vi "RDV-handle-AnalysePermittivityError.vi"(7 "%?":bool, 9 "set":i32, 10 "Reference key":string, 11 "RDV-Reflection_Data_viewer in":refnum<class "RDV-Reflection_Data_viewer.lvclass">) -> (0 "imag Error":dbl[](array[numeric]), 1 "imag":cluster{"Frequency":dbl[], "Perm 2":dbl[]}[](array[cluster]), 2 "real error":dbl[](array[numeric]), 3 "Real":cluster{"Frequency":dbl[], "Perm":dbl[]}[](array[cluster]))   [LabVIEW 2020, in "RDV-Reflection_Data_viewer.lvclass"]
doc: "Compares the permittivity of one data set in the viewer's map with the reference key, using RDC-permittivity-error_analysis. Returns the real and imaginary values and errors, as percent when %? is true."
uses:
  RDV-Reflection_Data_viewer.lvclass
  Computation/RDC-perm_calc_type.ctl
  RDV-Reflection_Data_viewer.lvclass/RDV-Reflection_Data_viewer.ctl
  Computation/RDC-Reflection_Data_Computation.lvlib
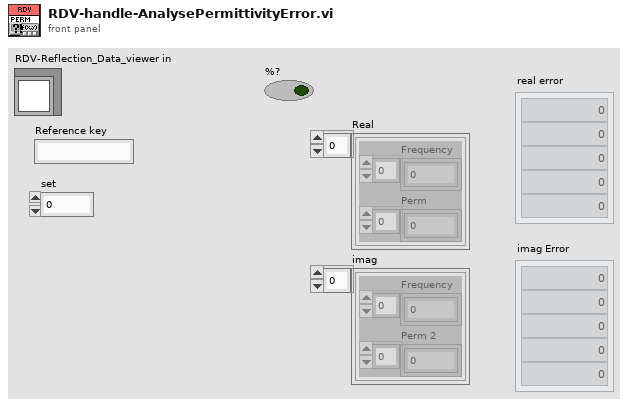
[diagram p1: front panel]
types:
  T1 = typedef "RDC-Reflection_Data_Computation.lvlib/RDC-perm_calc_type.ctl" = enum16{"Basic", "Capacative", "Advance", "Bilinear", "Size"}
  T2 = typedef "RDV-Reflection_Data_viewer.lvclass/RDV-UPDATE_IGNORE_LIST.ctl" = string[]
  T3 = typedef "RDV-Reflection_Data_viewer.lvclass/RDV-DATA_MAP.ctl" = map{string, T4}
  T4 = typedef "RDV-Reflection_Data_viewer.lvclass/RDV-DATA_MAP_CLUST.ctl" = cluster{"filename w/ ext":string, "Common Format":T5}
  T5 = typedef "RFH-Reflection_File_Handler.lvlib/RFH-common_data_format.ctl" = cluster{"Frequency":dbl[], "Reflection'":dbl[], "Reflection''":dbl[], "Permativity'":dbl[], "Permativity''":dbl[], "Conductivity":dbl[], "Loss Tangent":dbl[], "Resistance":dbl[], "Reactance":dbl[]}
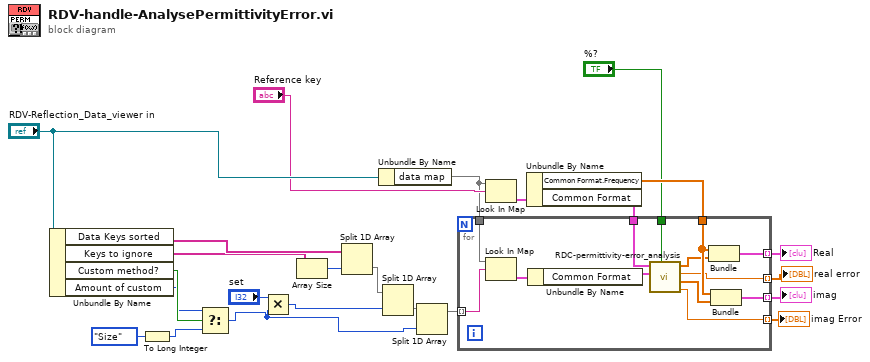
[diagram p0: block diagram]
diagram:
  n1 = Unbundle By Name("RDV-Reflection_Data_viewer in") -> ("Data Keys sorted"=w17:string[], "Keys to ignore"=w16:T2, "Custom method?"=w3:bool, "Amount of custom"=w2:i32)
  n2 = To Long Integer(number=RDC-perm_calc_type."Size" ("Perm calc type")) -> (32bit integer=w4:i32)
  n3 = Select(t=w2, s=w3, f=w4) -> (s? t:f=w1:i32)
  n4 = Multiply(x="set", y=w1) -> (x*y=w14:i32)
  n5 = Array Size(array=w16) -> (size(s)=w15:i32)
  n6 = Split 1D Array(array=w17, index=w15) -> (second subarray=w13:string[])  [unwired: 1 out]
  n7 = Unbundle By Name("RDV-Reflection_Data_viewer in") -> ("data map"=w21:T3)
  n8 = Split 1D Array(array=w13, index=w14) -> (second subarray=w12:string[])  [unwired: 1 out]
  n9 = Split 1D Array(array=w12, index=w1) -> (first subarray=w11:string[])  [unwired: 1 out]
  n10 = Look In Map(map=w21, key="Reference key") -> (value=w20:T4)  [unwired: 1 in, 1 out]
  n11 = Unbundle By Name(w20) -> ("Common Format.Frequency"=w18:dbl[], "Common Format"=w19:T5)
  n12 = for {
    tunnel: w21 -> [w34]
    tunnel: w19 -> [w37]
    tunnel: w18 -> [w36]
    tunnel: w11 -> [w33] mode=indexing
    tunnel: [w30] -> w10 mode=indexing
    tunnel: [w29] -> w9 mode=indexing
    tunnel: [w27] -> w8 mode=indexing
    tunnel: [w26] -> w7 mode=indexing
    tunnel: "%?" -> [w25]
    n13 = Look In Map(map=w34, key=w33) -> (value=w32:T4)  [unwired: 1 in, 1 out]
    n14 = Unbundle By Name(w32) -> ("Common Format"=w31:T5)
    n15 = call "RDC-permittivity-error_analysis.vi"("%?"=w25, "Analyse"=w31, "Correct"=w37) -> ("AVG imag"=w26:dbl, "Perm imag"=w35:dbl[], "AVG Real"=w27:dbl, "Perm real"=w28:dbl[])  [unwired: 5 in]
    n16 = Bundle("Frequency"=w36, "Perm real"=w28) -> (w30:cluster{"Frequency":dbl[], "Perm real":dbl[]})  [unwired: 1 in]
    n17 = Bundle("Frequency"=w36, "Perm imag"=w35) -> (w29:cluster{"Frequency":dbl[], "Perm imag":dbl[]})  [unwired: 1 in]
  }
  "Real" <- w10
  "imag" <- w9
  "real error" <- w8
  "imag Error" <- w7
